vi "Get sound from snd device.vi"(5 "init":bool, 6 "error in":errorcluster, 7 "Sound Rate":enum16{"11025", "22050", "44100"}(ring), 8 "buffer size (samples) : Ns":i32=8192 min=1024 step=1024, 9 "Input Sound device":i32) -> (0 "error out":errorcluster, 2 "sound out":dbl[](array[numeric]), 3 "task ID out":T1 format="%.0x")   [LabVIEW 2021]
doc: "The VI read sound from a Sound Device.\n\n::: CalcExpress Toolkit :::\nCopyright (c) 2000-2026 Konstantin Shifershteyn. All rights reserved."
uses:
  <vilib>/sound2/lvsound2.llb/Sound Input Task ID.ctl
  <vilib>/sound2/lvsound2.llb/Sound Data Format.ctl
  <vilib>/sound2/lvsound2.llb/Sampling Mode.ctl
  <vilib>/sound2/lvsound2.llb/Sound Input Read (DBL).vi
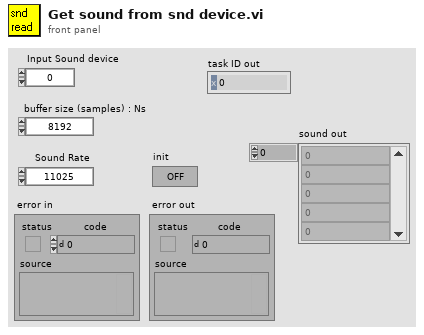
[diagram p1: front panel]
types:
  T1 = typedef "Sound Input Task ID.ctl" = u32
  T2 = typedef "Sound Data Format.ctl" = cluster{"sample rate (S/s)":dbl, "number of channels":i32, "bits per sample":i32}
  T3 = typedef "Sampling Mode.ctl" = i32
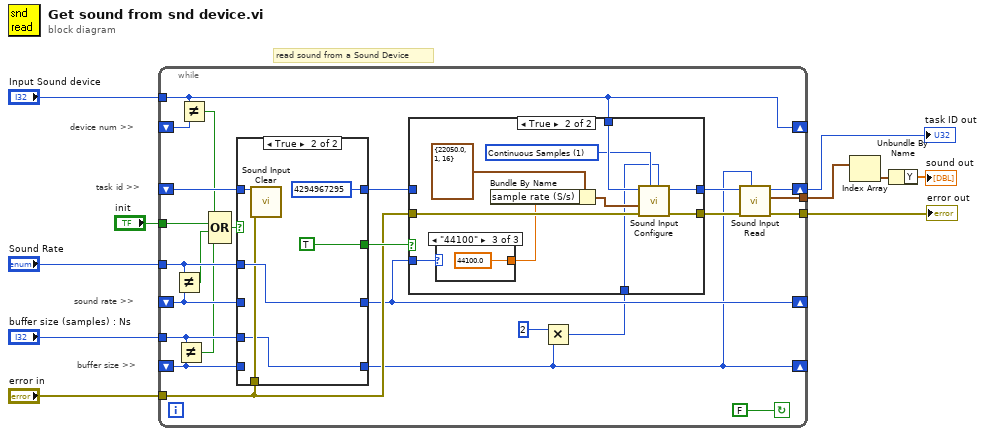
[diagram p0: block diagram]
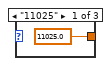
[diagram p3: hidden frame]
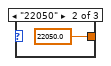
[diagram p4: hidden frame]
diagram:
  # "read sound from a Sound Device"
  # "buffer size >>"
  # "sound rate >>"
  # "task id >>"
  # "device num >>"
  n1 = while {
    tunnel: "init" -> [w19]
    tunnel: "buffer size (samples) : Ns" -> [w22]
    shift-left: _ -> [w21]
    shift-right: [w12] -> _
    tunnel: [w24] -> w7
    tunnel: "error in" -> [w27]
    tunnel: "Sound Rate" -> [w32]
    shift-left: _ -> [w34]
    shift-right: [w11] -> w1
    tunnel: "Input Sound device" -> [w17]
    shift-left: _ -> [w33]
    shift-right: [w23] -> _
    shift-left: _ -> [w35]
    shift-right: [w17] -> _
    tunnel: [w15] -> w4
    stop <- FALSE continue-if-true
    n2 = Not Equal?(x=w32, y=w33) -> (x != y?=w31:bool)
    n3 = Not Equal?(x=w22, y=w21) -> (x != y?=w20:bool)
    n4 = Not Equal?(x=w17, y=w35) -> (x != y?=w18:bool)
    n5 = Compound Arithmetic op=OR(w18, w19, w31, w20) -> (w30:bool)
    n6 = case shown="True" w30 {
      tunnel: w34 -> [w51 w58]
      tunnel: [w51 T1 4294967295 ("task ID out")] -> w28
      tunnel: [w53 w59] -> w23
      tunnel: w33 -> [w53 _]
      tunnel: w32 -> [_ w59]
      tunnel: [_ TRUE] -> w29
      tunnel: w27 -> [_ w56]
      tunnel: w21 -> [w52 _]
      tunnel: [w52 w55] -> w12
      tunnel: w22 -> [_ w55]
      frame False {
      }
      frame True {
        n7 = call <vilib>:"Sound Input Clear.vi"("error in (no error)"=w56, "task ID"=w58) -> ()  [unwired: 9 in, 1 out]
      }
    }
    n8 = Multiply(x=2, y=w12) -> (x*y=w13:i32)
    n9 = case shown="True" w29 {
      tunnel: w28 -> [w37 _]
      tunnel: [w37 w39] -> w26
      tunnel: w17 -> [_ w47]
      tunnel: w27 -> [w36 w46]
      tunnel: [w36 w38] -> w25
      tunnel: w23 -> [_ w43]
      tunnel: w13 -> [_ w40]
      frame False {
      }
      frame True {
        w41 = T3 1 items=["Finite Samples", "Continuous Samples"] ("sample mode")
        n10 = case shown="\"44100\"" w43 {
          tunnel: [11025.0 22050.0 44100.0] -> w42
          frame "11025" {
          }
          frame "22050" {
          }
          frame "44100" {
          }
        }
        n11 = Bundle By Name(cluster=T2 {"sample rate (S/s)"=22050.0, "number of channels"=1, "bits per sample"=16} ("sound format"), "sample rate (S/s)"=w42) -> (w44:T2)
        n12 = call <vilib>:"Sound Input Configure.vi"("number of samples/ch"=w40, "sample mode"=w41, "error in (no error)"=w46, "sound format"=w44, "device ID"=w47) -> ("error out"=w38:errorcluster, "task ID"=w39:T1)  [unwired: 5 in]
      }
    }
    n13 = call-poly <vilib>:"Sound Input Read.vi"("number of samples/ch"=w12, "error in (no error)"=w25, "task ID"=w26) -> ("error out"=w24:errorcluster, "data"=w15:waveform(dbl)[], "task ID out"=w11:T1)  [unwired: 6 in]
  }
  "error out" <- w7
  "task ID out" <- w1
  n14 = Index Array(array=w4) -> (element=w3:waveform(dbl))  [unwired: 1 in]
  n15 = Unbundle By Name(w3) -> ("Y"=→"sound out":dbl[])
